vi "Sim_Fault_Injection.vi"(8 "error in (no error)":errorcluster={"status"=FALSE, "code"=0, "source"="\"\""}, 10 "trigger condition/time":string, 11 "Fault type":string) -> (0 "error out":errorcluster={"status"=FALSE, "code"=0, "source"="\"\""}, 2 "status ok":bool, 3 "Modified device/transport behavior":string)   [LabVIEW 2026]
doc: "INTENT: Inject repeatable failure scenarios. LOGIC: Introduce sensor stale/dropout, lost ACK, stuck servo, saturation, plugin stall, Host disconnect and disk full."
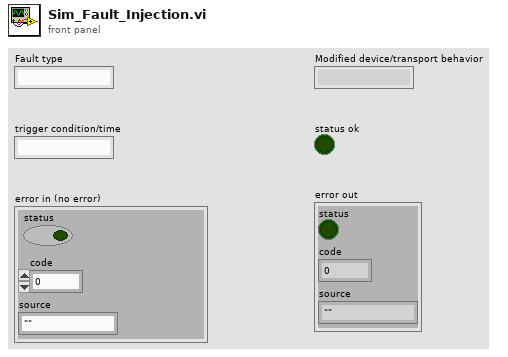
[diagram p1: front panel]
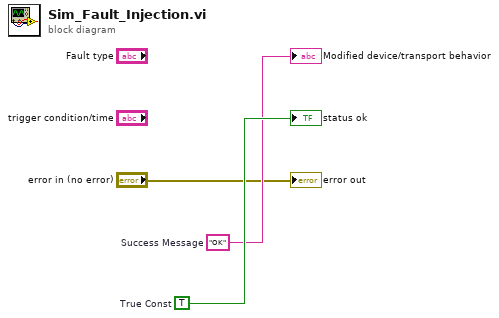
[diagram p0: block diagram]
diagram:
  w3 = TRUE  # True Const
  w2 = "OK"  # Success Message
  "Modified device/transport behavior" <- w2
  "status ok" <- w3
  "error out" <- "error in (no error)"
